vi "LTE check RB Status.vi"(8 "error in (no error)":errorcluster caption="에러 입력(에러 없음)", 10 "RB Offset":i32, 11 "Instrument Manager 입력":refnum<class "Instrument Manager.lvclass">) -> (0 "error out":errorcluster caption="에러 출력", 2 "불리언":bool, 3 "Instrument Manager 출력":refnum<class "Instrument Manager.lvclass">)   [LabVIEW 2023, in "Instrument Manager.lvclass"]
uses:
  Instrument Manager.lvclass
  Instrument Manager.lvclass/Instrument Manager.ctl
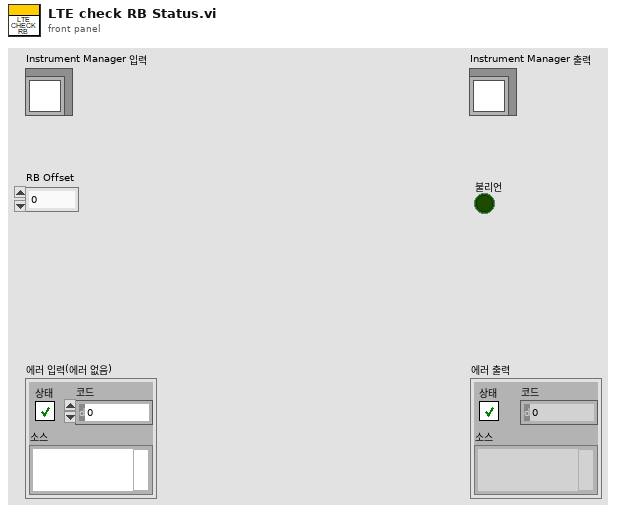
[diagram p1: front panel]
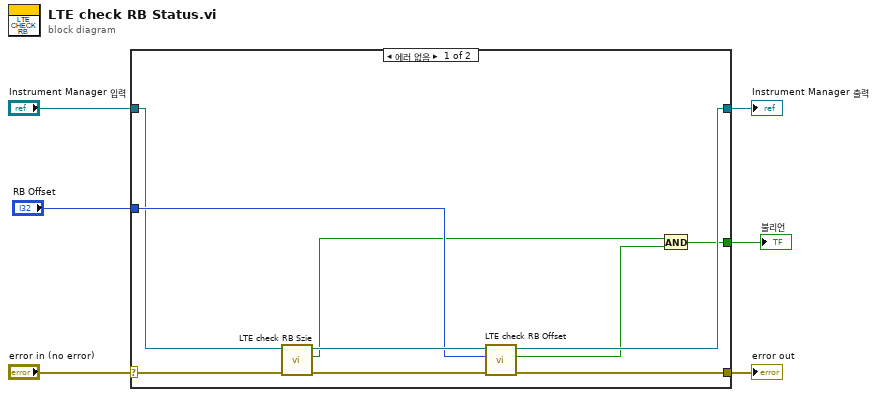
[diagram p0: block diagram]
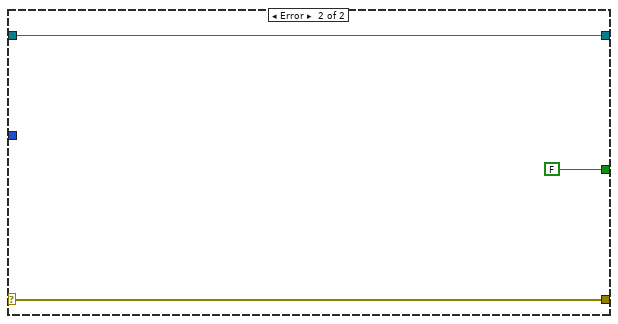
[diagram p2: hidden frame]
diagram:
  n1 = case shown="에러 없음" "error in (no error)" {
    selector: "error in (no error)" -> [w16 w19]
    tunnel: [w14 w19] -> w5
    tunnel: [w10 w18] -> w3
    tunnel: "Instrument Manager 입력" -> [w11 w18]
    tunnel: "RB Offset" -> [w12 _]
    tunnel: [w7 FALSE] -> w1
    frame No Error {
      n2 = call "LTE check RB Szie.vi"("error in (no error)"=w16, "Instrument Manager 입력"=w11) -> ("error out"=w15:errorcluster, "불리언"=w8:bool, "Instrument Manager 출력"=w13:refnum<class "Instrument Manager.lvclass">)  [unwired: 7 in]
      n3 = call "LTE check RB Offset.vi"("error in (no error)"=w15, "RB Offset"=w12, "Instrument Manager 입력"=w13) -> ("error out"=w14:errorcluster, "불리언"=w9:bool, "Instrument Manager 출력"=w10:refnum<class "Instrument Manager.lvclass">)  [unwired: 6 in]
      n4 = And(x=w8, y=w9) -> (x .and. y?=w7:bool)
    }
    frame Error {
    }
  }
  "error out" <- w5
  "Instrument Manager 출력" <- w3
  "불리언" <- w1
